vi "W13_Judge_Washer.vi"() -> ()   [LabVIEW 2018]
doc: "Use this template to build a VI to use as a subVI."
panel:
  out "OK":bool
  in  "area ratio":dbl
  out "diameter mm":dbl
  in  "px per mm":dbl
  in  "outer width px":dbl
  # "Try first: outer width 161 px, 8.1 px per mm, area ratio 0.99 -> 19.88 mm, OK. All zeros give 0/0 = NaN."
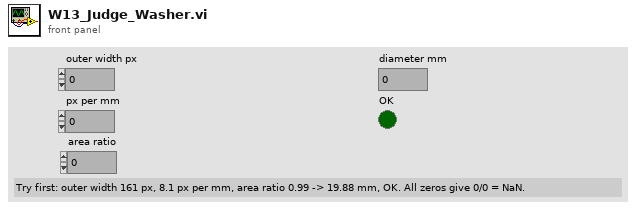
[diagram p1: front panel]
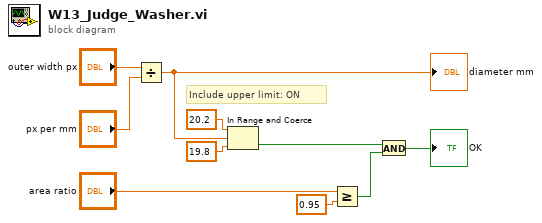
[diagram p0: block diagram]
diagram:
  # "Include upper limit: ON"
  n1 = Divide(x="outer width px", y="px per mm") -> (x/y=w8:dbl)
  "diameter mm" <- w8
  n2 = In Range and Coerce(upper limit=20.2, x=w8, lower limit=19.8) -> (In Range?=w3:bool)  [unwired: 1 out]
  n3 = Greater Or Equal?(x="area ratio", y=0.95) -> (x >= y?=w2:bool)
  n4 = And(x=w3, y=w2) -> (x .and. y?=→"OK":bool)
